vi "IToolFGV.vi"(10 "Action":enum16{"GET", "SET"}(ring), 11 "ITool.lvclass in":refnum<class "ITool.lvclass">) -> (3 "ITool.lvclass out":refnum<class "ITool.lvclass">)   [LabVIEW 2017]
uses:
  Server/ITool/ITool.lvclass
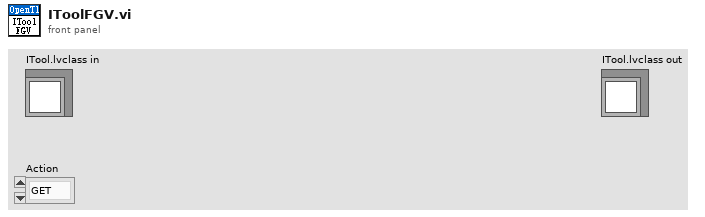
[diagram p1: front panel]
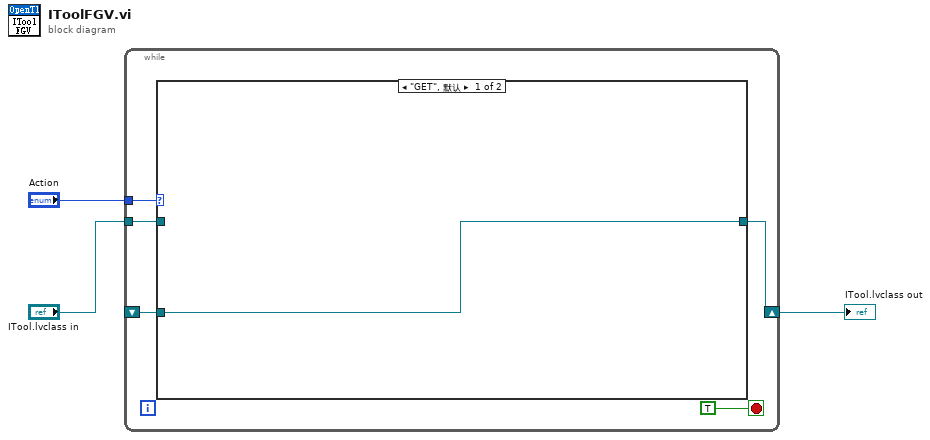
[diagram p0: block diagram]
diagram:
  n1 = while {
    shift-right: [w5] -> w3
    shift-left: _ -> [w4]
    tunnel: "Action" -> [w7]
    tunnel: "ITool.lvclass in" -> [w6]
    stop <- TRUE stop-if-true
    n2 = case shown="\"GET\", 默认" w7 {
      tunnel: w6 -> [_ w10]
      tunnel: [w9 w10] -> w5
      tunnel: w4 -> [w9 _]
      frame "GET", Default {
      }
      frame "SET" {
      }
    }
  }
  "ITool.lvclass out" <- w3
